vi "A_Loop.vi"(0 "Numeric":i32, 1 "N per point":i32=1, 3 "Tset setting":dbl, 5 "Numeric 2":i32, 7 "instrument handle out":refnum<k15>, 9 "Numeric 3":i32, 11 "Numeric 4":dbl, 12 "x":dbl) -> (4 "Averaged":string[](array[string]), 8 "Frequency":string[](array[string]), 10 "Unaveraged":string[](array[string]), 14 "Averaged2":string[](array[string]), 15 "Frequency2":string[](array[string]))   [LabVIEW 2025]
panel:
  out "error out":errorcluster
  out "Progress":dbl(slide) scale=0.1..100.0
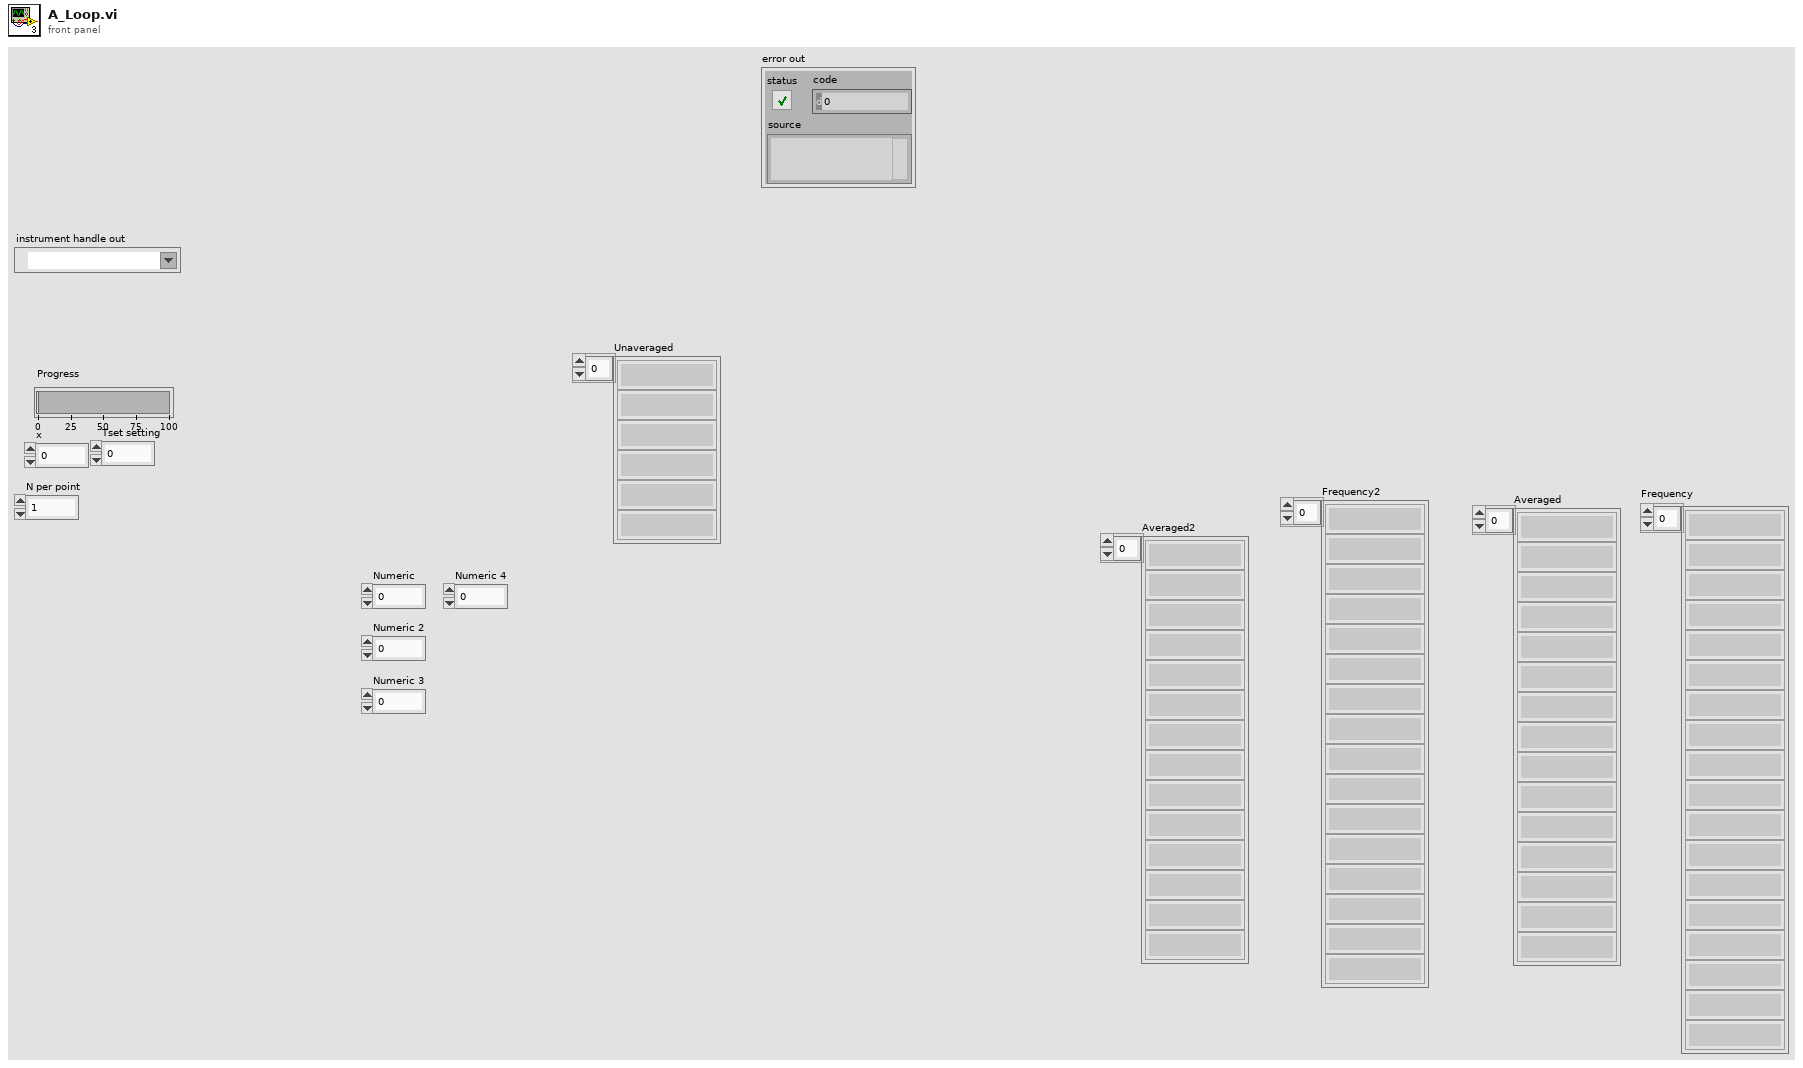
[diagram p1: front panel]
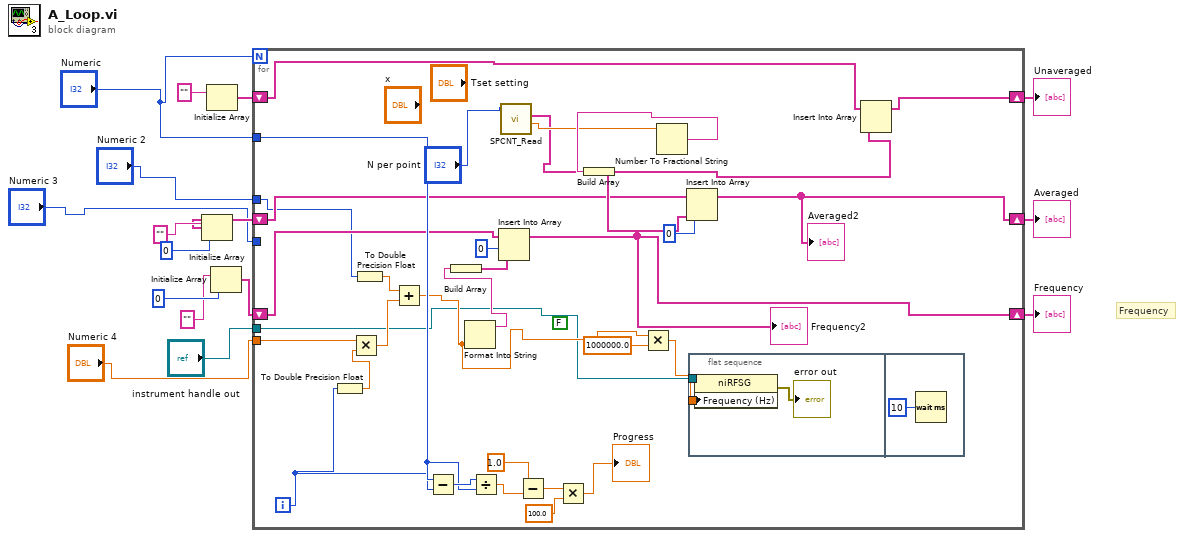
[diagram p0: block diagram]
diagram:
  # "Frequency"
  n1 = Initialize Array("", 0 ("dimension size")) -> (w12:string[])
  n2 = Initialize Array("") -> (w3:string[])  [unwired: 1 in]
  n3 = Initialize Array("", 0 ("dimension size")) -> (w11:string[])
  n4 = for {
    N: "Numeric" -> [_]
    tunnel: "Numeric 4" -> [w48]
    tunnel: "Numeric 2" -> [w28]
    tunnel: "Numeric" -> [w41]
    tunnel: "Numeric 3" -> [_]
    shift-right: [w30] -> w10
    shift-left: w12 -> [w32]
    shift-right: [w33] -> w9
    shift-left: w11 -> [w31]
    shift-right: [w26] -> w2
    shift-left: w3 -> [w27]
    tunnel: "instrument handle out" -> [w18]
    i -> [w21]
    (unwired) FALSE ("First time?")
    n5 = To Double Precision Float(number=w21) -> (double precision float=w47:dbl)
    n6 = Multiply(x=w48, y=w47) -> (x*y=w34:dbl)
    n7 = To Double Precision Float(number=w28) -> (double precision float=w35:dbl)
    n8 = Add(x=w35, y=w34) -> (x+y=w19:dbl)
    n9 = Subtract(x=w41, y=w21) -> (x-y=w42:i32)
    n10 = Format Into String(w19) -> (resulting string=w25:string)  [unwired: 3 in, 1 out]
    n11 = Build Array(w25) -> (w46:string[])
    n12 = Divide(x=w42, y=w41) -> (x/y=w39:dbl)
    n13 = Insert Into Array "Insert Into Array"(array=w31, index=0 ("index (row)"), new element=w46) -> (w33:string[])
    "Frequency2" <- w33
    n14 = call "SPCNT_Read.vi"("N per point"="N per point") -> ("x/y"=w23:dbl, "Array"=w22:string[])  [unwired: 9 in]
    n15 = Subtract(x=1.0, y=w39) -> (x-y=w38:dbl)
    n16 = Multiply(x=w38, y=100.0) -> (x*y=→"Progress":dbl)
    n17 = Multiply(x=w19, y=1000000.0) -> (x*y=w17:dbl)
    n18 = Number To Fractional String(number=w23) -> (F-format string=w36:string)  [unwired: 3 in]
    n19 = Build Array(w36) -> (w44:string[])
    n20 = Insert Into Array "Insert Into Array"(array=w32, index=0, new element=w44) -> (w30:string[])
    "Averaged2" <- w30
    n21 = flat-sequence {
      tunnel: w18 -> [w51]
      tunnel: w17 -> [w50]
      frame #0 {
        n22 = property class="niRFSG"(reference=w51, "Frequency (Hz)"=w50) -> (error out=→"error out":errorcluster)  [unwired: 1 in, 1 out]
      }
      frame #1 {
        n23 = Wait (ms)(milliseconds to wait=u32 10) -> ()  [unwired: 1 out]
      }
    }
    n24 = Insert Into Array(array=w27, new element=w22) -> (w26:string[])  [unwired: 1 in]
  }
  "Averaged" <- w10
  "Frequency" <- w9
  "Unaveraged" <- w2
